vi "温度采集 - TP1.vi"(7 "CSM Name":string="TP1") -> ()   [LabVIEW 2026, in "UI-温度采集.lvlib"]
uses:
  Supports/Sample Settings.ctl
  Supports/Ch Settings.ctl
  Data ColndSave/Supports/Time and Data.ctl
  <userlib>/_NEVSTOP/Communicable State Machine(CSM)/_Polymophic/CSM - Filter Duplicated Lines.vi
  65d0c194-c74c-4b0e-a0ba-0dceafb13ea2.vi
  a3283b4f-3d7d-475f-8286-b95f18be6a9d.vi
  5ee6f246-6564-45f2-9b1c-adf21ebee76f.vi
  67e6e356-fdb8-4529-b23b-6ce46d2feb59.vi
  c25498cf-601b-4c58-9055-343fcb9f8f4a.vi
  c6692627-02fb-4556-9c5d-59e6097d0856.vi
  8c0fc226-3871-4866-9b38-f175316b3ef9.vi
  <vilib>/Analysis/baseanly.llb/Mean (DBL).vi
  f7ac7929-c03e-4c45-8e54-d37ffbbe8d04.vi
  8417ea6c-3bd9-4cd5-8933-b29b0935beb3.vi
  c0a7cae7-a94b-4088-a6e9-4f476a10c4ba.vi
  <userlib>/_NEVSTOP/Communicable State Machine(CSM)/_Polymophic/CSM - Replace Marks in Messages.vi
  5163a33a-69e0-492d-a74e-a390bdb1a610.vi
  ba09a988-f7d6-44f3-a6d8-47fd2b4ee3b5.vi
  7fbb40cc-7bce-4797-8461-cf694f50c740.vi
  2b068055-2750-46ca-adeb-001e26472588.vi
  <userlib>/_NEVSTOP/Communicable State Machine(CSM)/AdvanceAPI/CSM - Compact Multiple States.vi
  <userlib>/_NEVSTOP/Communicable State Machine(CSM)/AdvanceAPI/CSM - Break Down Multiple States String.vi
  <userlib>/_NEVSTOP/Communicable State Machine(CSM)/_Shared/Remove Comments from Single-line.vi
  <userlib>/_NEVSTOP/Communicable State Machine(CSM)/_Shared/Split Single-line Message.vi
  <userlib>/_NEVSTOP/Communicable State Machine(CSM)/_Shared/Trim Single-line Text.vi
  <userlib>/_NEVSTOP/Communicable State Machine(CSM)/AdvanceAPI/CSM - Revert Arguments-Safe String.vi
  <userlib>/_NEVSTOP/Communicable State Machine(CSM)/AdvanceAPI/CSM - Make String Arguments Safe.vi
  c25498cf-601b-4c58-9055-343fcb9f8f4a.vi/99de0c97-112a-4c86-9094-c187659127e1.vi
  <userlib>/_NEVSTOP/Communicable State Machine(CSM)/Utility/Build Error Cluster.vi
  c6692627-02fb-4556-9c5d-59e6097d0856.vi/99de0c97-112a-4c86-9094-c187659127e1.vi
  f7ac7929-c03e-4c45-8e54-d37ffbbe8d04.vi/99de0c97-112a-4c86-9094-c187659127e1.vi
  8417ea6c-3bd9-4cd5-8933-b29b0935beb3.vi/99de0c97-112a-4c86-9094-c187659127e1.vi
  <userlib>/_NEVSTOP/Communicable State Machine(CSM)/AdvanceAPI/CSM - Keywords.vi
  <userlib>/_NEVSTOP/Communicable State Machine(CSM)/addons/API-String-Arugments-Support/_Support/Data To API String Arguments.vi
  <userlib>/_NEVSTOP/Communicable State Machine(CSM)/addons/INI-Static-Variable-Support/_Support/instances/_CSM - Read File Logger Configuration - v1.0.vi
  <vilib>/Utility/Data Type/Get Type Information.vi
  <userlib>/_NEVSTOP/Communicable State Machine(CSM)/addons/API-String-Arugments-Support/_Support/Data To SingleElementsArray_csm.vi
  <userlib>/_NEVSTOP/Communicable State Machine(CSM)/addons/INI-Static-Variable-Support/_Support/Parse Used Session and Name.vi
  <userlib>/_NEVSTOP/Communicable State Machine(CSM)/addons/INI-Static-Variable-Support/_Support/INI-FGV(lvlibp).vi
  <userlib>/_NEVSTOP/Communicable State Machine(CSM)/addons/INI-Static-Variable-Support/_Support/Populate String with INI Variable.vi
  <userlib>/_NEVSTOP/Communicable State Machine(CSM)/addons/API-String-Arugments-Support/_Support/Convert API String Arguments to Data(variant).vi
  <userlib>/_NEVSTOP/Communicable State Machine(CSM)/addons/API-String-Arugments-Support/_Support/SingleElementsArray To Data_csm.vi
  <userlib>/_NEVSTOP/Communicable State Machine(CSM)/addons/MassData-Parameter/_support/FGV-MassData(lvlibp).vi
  <userlib>/_NEVSTOP/Communicable State Machine(CSM)/Communicable State Machine.lvlib
  <vilib>/Analysis/NI_AALBase.lvlib
  Acquisition/Acquisition.lvlib
  <userlib>/_NEVSTOP/Communicable State Machine(CSM)/addons/MassData-Parameter/CSM MassData Parameter Support.lvlib
  <userlib>/_NEVSTOP/Communicable State Machine(CSM)/addons/INI-Static-Variable-Support/INI-Static-Variable-Support.lvlib
  <userlib>/_NEVSTOP/Communicable State Machine(CSM)/addons/Watchdog/CSM Watchdog.lvlib
  <userlib>/_NEVSTOP/Communicable State Machine(CSM)/addons/Logger/CSM File Logger.lvlib
  Logging/Logging.lvlib
  Data ColndSave/Data Collection and Save.lvlib
panel:
  in  "停止":bool
  in  "温度显示":T1(tab)
  in  "温度采集开关":bool
  in  "Offset relative to chX":T2(ring)
  out "Final Temp":dbl[](array[numeric]) format="%#.2g"
  in  "USB Port":refnum<visa-resource-name>="COM3"
  in  "Interval(s)":dbl=0.5
  in  "Calib":dbl[](array[numeric])=[0.0, 0.0, 0.0, 0.0, 0.0, 0.0, 0.0, 0.0]
  out "Offset":dbl[](array[numeric]) format="%#.2g"
  in  "Chart Auto Zoom":bool=TRUE
  in  "ChA":T3
  in  "ChB":T3
  in  "ChC":T3
  in  "ChD":T3
  out "Default 2":waveform(dbl)(graph)
  out "Default 1":waveform(dbl)(graph)
  out "Default 4":waveform(dbl)(graph)
  out "Default 3":waveform(dbl)(graph)
  out "Default 6":waveform(dbl)(graph)
  out "Default 5":waveform(dbl)(graph)
  out "Default 8":waveform(dbl)(graph)
  out "Default 7":waveform(dbl)(graph)
  out "Diff 2 (CHC-CHD)":waveform(dbl)(graph)
  out "DIff 1 (ChA-CHB)":waveform(dbl)(graph)
  in  "子程序？":bool
  out "Error Occurred":errorcluster caption="温度采集-错误输出"
  out "State History":string
  # "-"
  # "-"
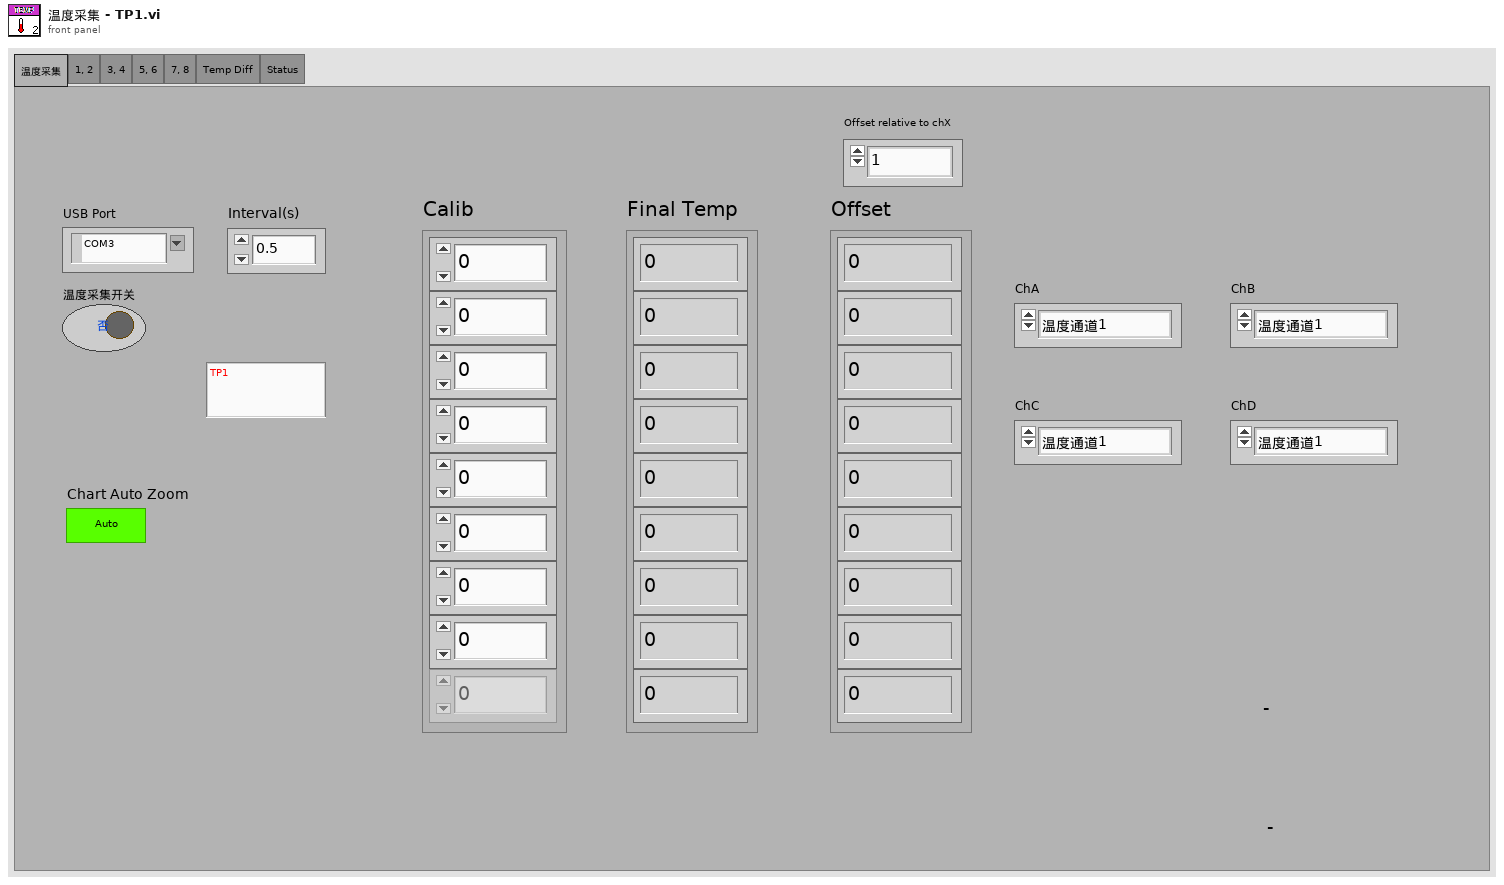
[diagram p1: front panel]
types:
  T1 = enum32{"温度采集", "1, 2", "3, 4", "5, 6", "7, 8", "Temp Diff", "Status"}
  T2 = enum16{"1", "2", "3", "4", "5", "6", "7", "8", "中值", "平均值"}
  T3 = typedef "温度通道索引_全局.ctl" = enum16{"温度通道1", "温度通道2", "温度通道3", "温度通道4", "温度通道5", "温度通道6", "温度通道7", "温度通道8", "TC1控制温度", "TC1实际温度", "TC1实际输出电压", "TC1实际输出电流", "TC1实际输出功率", "TC2控制温度", "TC2实际温度", "TC2实际输出电压", "TC2实际输出电流", "TC2实际输出功率", "压力(电压值)", "压力(g)", "Zolix当前位置", "Zolix速度", "步进电机位置", "步进电机速度", "温度", "湿度"}
  T4 = cluster{"Enable":bool, "Limit":cluster{"FileSize":i64, "FileNum":i32}, "Timestamp.Format":string, "AutoExit":bool}
  T5 = enum32{"Invalid", "Standard", "Closed", "Hidden", "Minimized", "Maximized"}
  T6 = enum32{"invalid app kind", "Development System", "Run Time System", "Student Edition", "Embedded LabVIEW", "Evaluation", "Custom"}
  T7 = typedef "Communicable State Machine.lvlib/_CSM_Response Source Message.ctl" = cluster{"‘State":string, "’Arguments":string, "’Error":errorcluster}
  T8 = cluster{"Current VI Reference":refnum<vi>, "Close Panel on Exit?":bool}
  T9 = typedef "UI-温度采集.lvlib/Sample Settings.ctl" = cluster{"USB Port":refnum<visa-resource-name>, "Interval(s)":dbl, "Calib":dbl[]}
  T10 = typedef "Data Collection and Save.lvlib/Time and Data.ctl" = cluster{"采集时间":timestamp, "Data":dbl[]}
  T11 = cluster{"Core":cluster{"Current VI Reference":refnum<vi>, "Close Panel on Exit?":bool}, "Sample Settings":T9, "Time and Data":T10, "子程序？":bool}
  T12 = typedef "UI-温度采集.lvlib/Ch Settings.ctl" = cluster{"Offset relative to chX":enum16{"1", "2", "3", "4", "5", "6", "7", "8", "中值", "平均值"}, "ChA":T3, "ChB":T3, "ChC":T3, "ChD":T3}
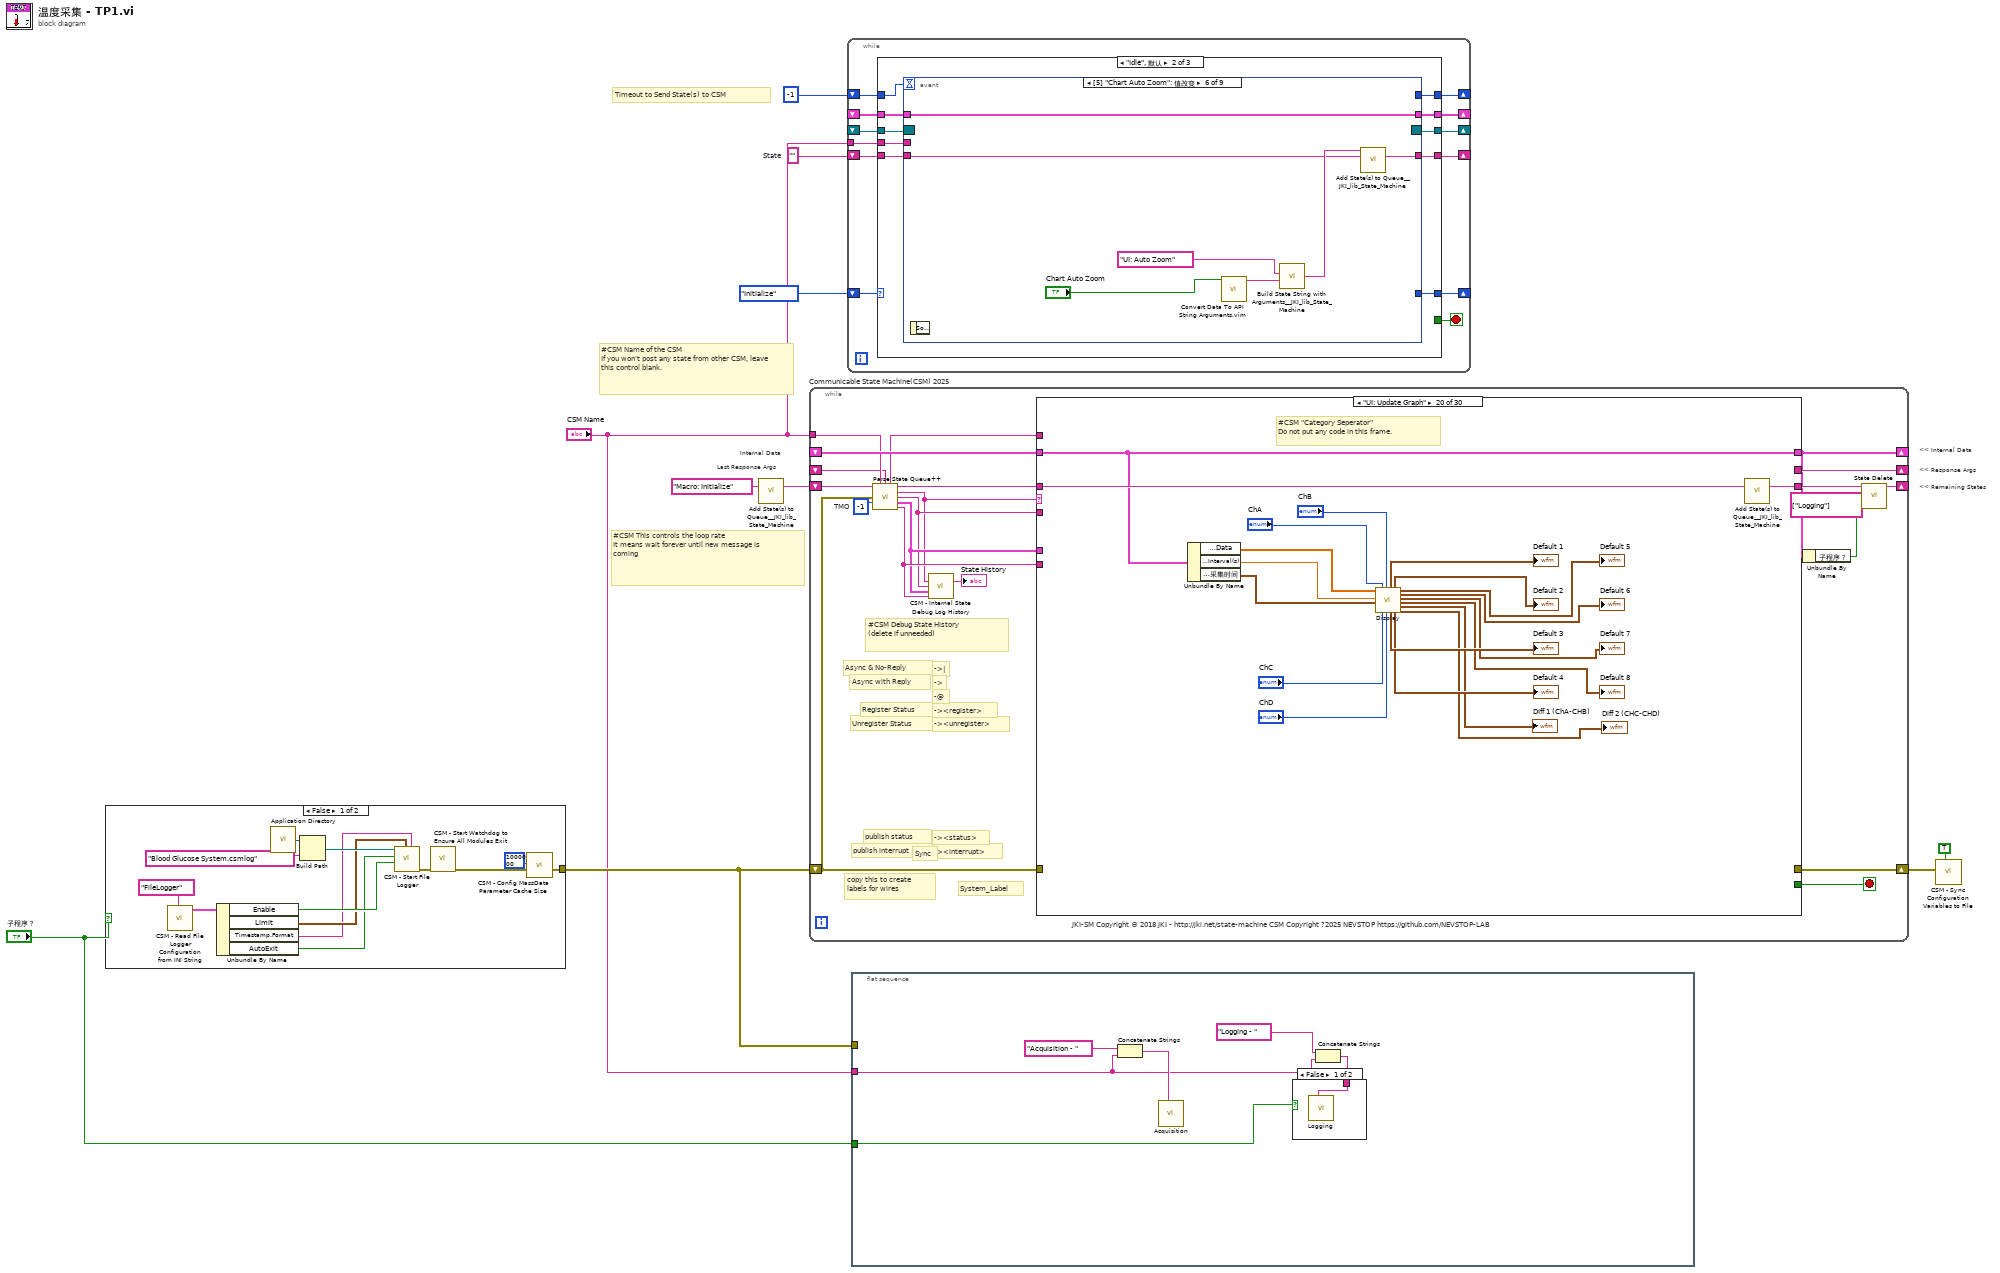
[diagram p0: block diagram]
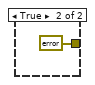
[diagram p2: hidden frame]
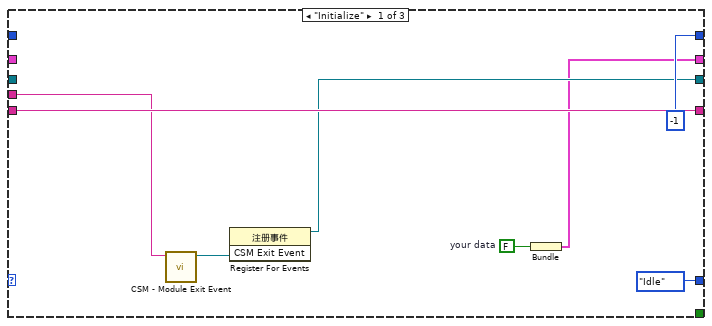
[diagram p4: hidden frame]
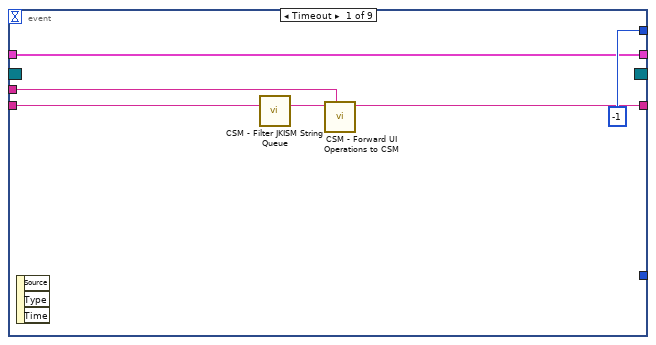
[diagram p5: hidden frame]
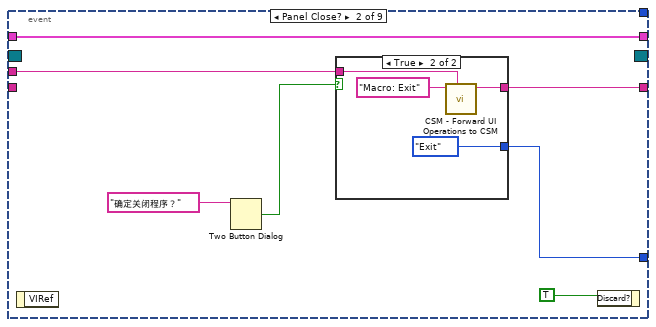
[diagram p6: hidden frame]
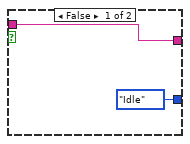
[diagram p7: hidden frame]
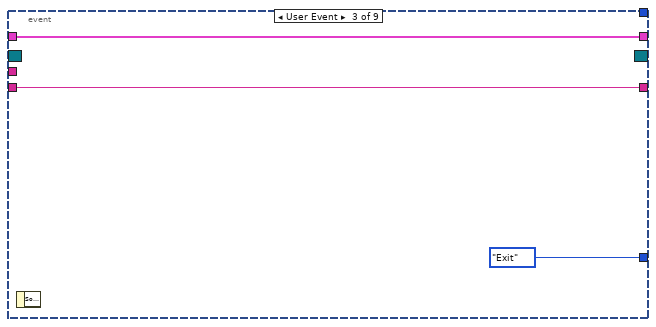
[diagram p8: hidden frame]
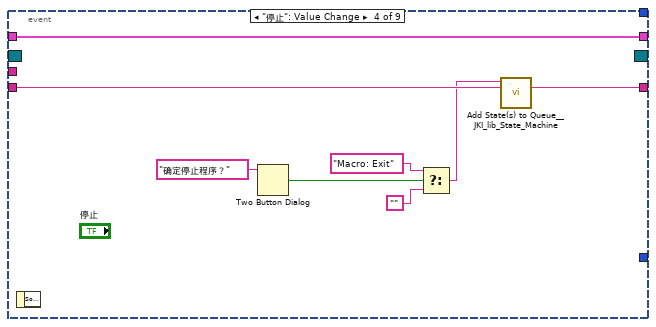
[diagram p9: hidden frame]
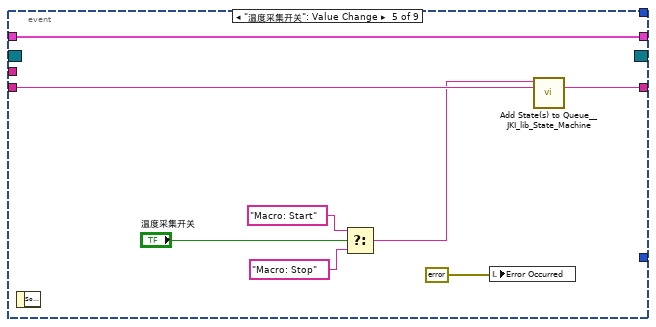
[diagram p10: hidden frame]
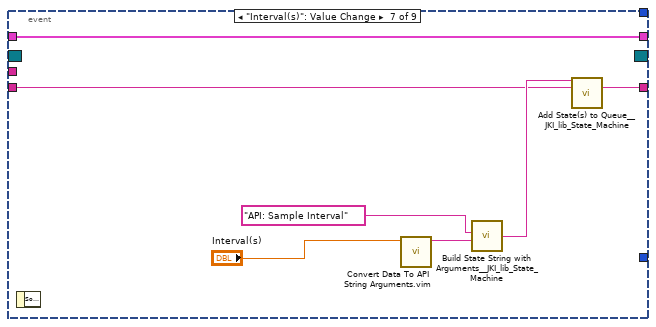
[diagram p11: hidden frame]
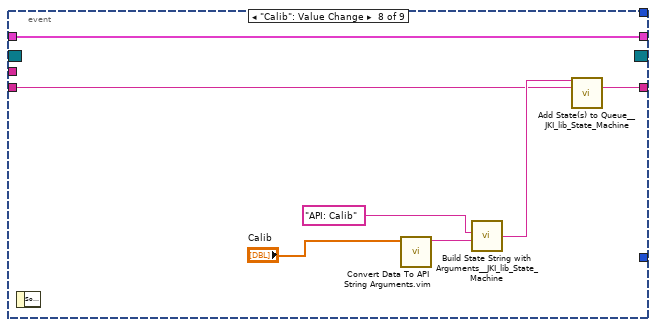
[diagram p12: hidden frame]
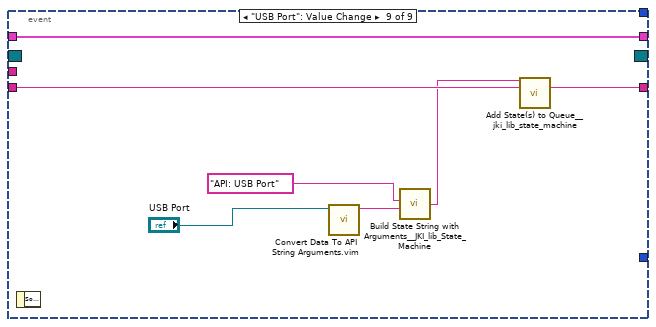
[diagram p13: hidden frame]
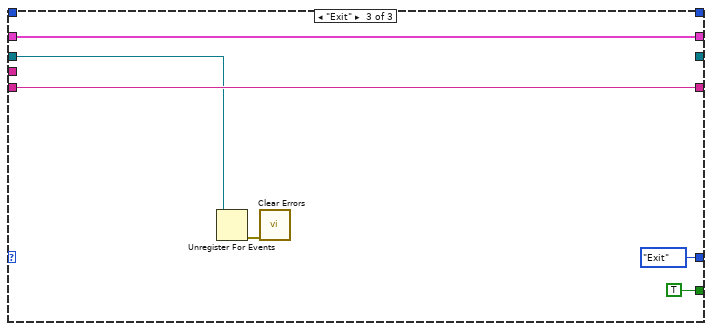
[diagram p14: hidden frame]
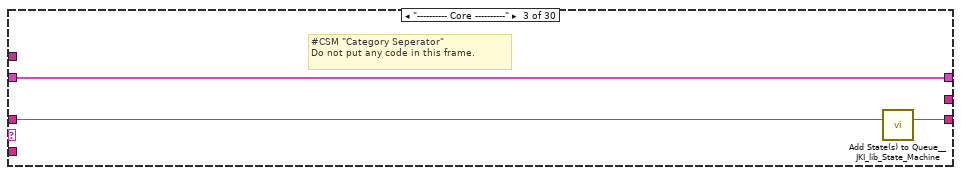
[diagram p17: hidden frame]
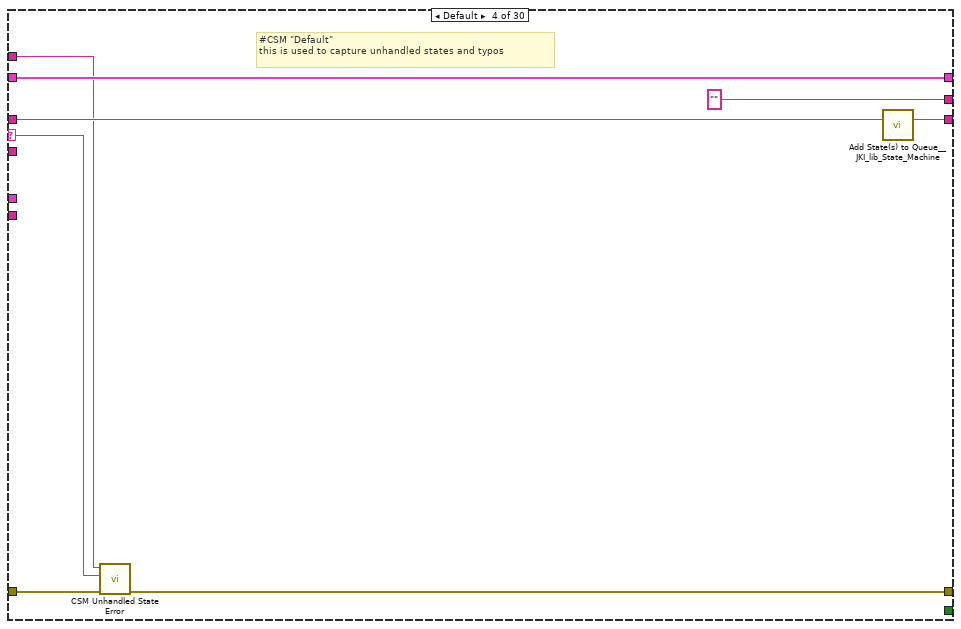
[diagram p18: hidden frame]
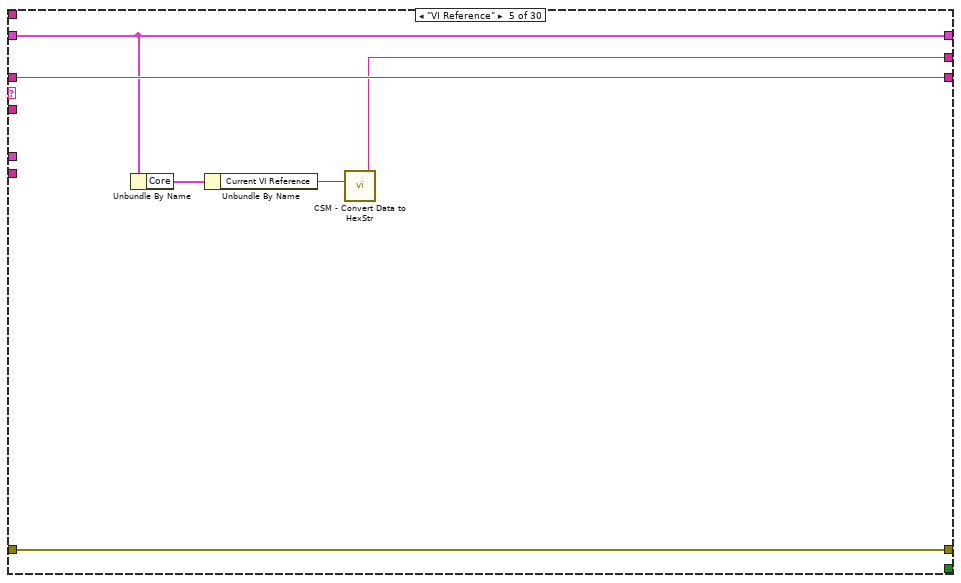
[diagram p19: hidden frame]
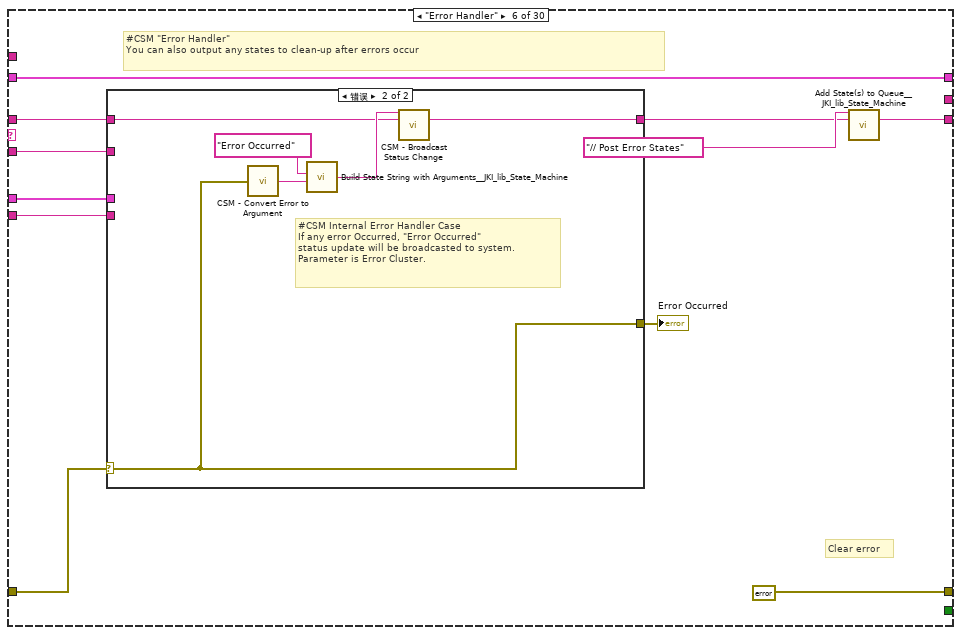
[diagram p20: hidden frame]
diagram:
  w9 = ""  # State
  # "Timeout to Send State(s) to CSM"
  # "Last Response Args"
  # "Internal Data"
  # "#CSM Name of the CSM\nIf you won't post any state from other CSM, leave this control blank."
  # "#CSM This controls the loop rate\nIt means wait forever until new message is coming"
  # "<< Internal Data"
  # "<< Response Args"
  # "<< Remaining States"
  n1 = case shown="False" "子程序？" {
    tunnel: [w11 errorcluster {"status"=FALSE, "code"=0, "source"=""} ("Error out")] -> w5
    frame False {
      n2 = call-poly <userlib>:"CSM - Read File Logger Configuration from INI String.vi"("Section Name(\"FileLogger\")"="FileLogger" ("Section Name(\"\" as Default)")) -> ("FileLogger Configuration-v1"=w18:T4)  [unwired: 7 in, 1 out]
      n3 = Unbundle By Name(w18) -> ("Enable"=w17:bool, "Limit"=w16:cluster{"FileSize":i64, "FileNum":i32}, "Timestamp.Format"=w14:string, "AutoExit"=w15:bool)
      n4 = call <vilib>:"Application Directory.vi"() -> ("Application Directory"=w23:path)
      n5 = Build Path(base path=w23, name or relative path="Blood Glucose System.csmlog") -> (appended path=w21:path)
      n6 = call <userlib>:"CSM - Start File Logger.vi"("Timestamp Format"=w14, "Log Limit"=w16, "Watchdog? (T)"=w17, "Exit When All Module Exist? (F)"=w15, "Log File Path"=w21) -> ("error out"=w20:errorcluster)  [unwired: 4 in, 2 out]
      n7 = call <userlib>:"CSM - Start Watchdog to Ensure All Modules Exit.vi"("error in (no error)"=w20) -> ("error out"=w12:errorcluster)  [unwired: 10 in]
      n8 = call <userlib>:"CSM - Config MassData Parameter Cache Size.vi"("Error in"=w12, "Size (50M)"=1000000 ("size(1M)")) -> ("Error out"=w11:errorcluster)  [unwired: 9 in]
    }
    frame True {
    }
  }
  n9 = call <vilib>:"Add State(s) to Queue__JKI_lib_State_Machine.vi"("State(s) in (\"\")"="Macro: Initialize" ("Init State(\"Macro: Initialize\")")) -> ("States Out"=w6:string)  [unwired: 14 in]
  n10 = while "Communicable State Machine(CSM) 2025" {
    shift-right: [w26] -> _
    shift-left: _ -> [w41]
    shift-right: [w43] -> w3
    shift-left: w5 -> [w31]
    shift-right: [w28] -> _
    shift-left: w6 -> [w44]
    tunnel: "CSM Name" -> [w38]
    shift-right: [w39] -> _
    shift-left: _ -> [w33]
    stop <- w42 stop-if-true
    w40 = -1  # TMO
    # "#CSM Debug State History\n(delete if unneeded)"
    # "-><interrupt>"
    # "-><status>"
    # "-><unregister>"
    # "-><register>"
    # "-@"
    # "->"
    # "->|"
    # "publish interrupt"
    # "publish status"
    # "Unregister Status"
    # "Register Status"
    # "Sync"
    # "Async with Reply"
    # "Async & No-Reply"
    # "JKI-SM Copyright © 2018 JKI - http://jki.net/state-machine CSM Copyright ?2025 NEVSTOP https://github.com/NEVSTOP-LAB"
    # "copy this to create labels for wires"
    # "System_Label"
    n11 = call <userlib>:"Parse State Queue++.vi"("State Queue"=w44, "Name (\"\" to Use UUID)"=w38, "Response Arguments"=w33, "Previous Error"=w31, "Dequeue (1 ms)"=w40) -> ("Name Used"=w32:string, "Remaining States"=w45:string, "Current State"=w34:string, "Arguments"=w35:string, "Additional Information"=w36:T7, "Source CSM"=w37:string)  [unwired: 5 in]
    n12 = call <userlib>:"CSM - Internal State Debug Log History.vi"("State"=w34, "Arguments (\"\")"=w35, ">> Response Source Message >>"=w36, "Source (\"\")"=w37) -> ("Debug Log"=→"State History":string)  [unwired: 11 in]
    n13 = case shown="\"UI: Update Graph\"" w34 {
      selector: w34 -> [_ _ _ w56 _ _ _ _ _ _ _ _ _ _ _ _ _ _ _ _ _ _ _ _ _ _ _ _ _ _]
      tunnel: w45 -> [w46 w49 w52 w60 w65 w71 w96 w102 w108 w118 w125 w137 w141 w144 w164 w176 w223 w226 w237 w257 w264 w269 w275 w284 w291 w297 w300 w311 w321 w328]
      tunnel: w35 -> [_ _ _ _ _ w70 w92 w99 w105 w112 _ _ _ _ _ w171 _ _ _ _ w260 _ _ _ _ _ _ w306 w314 w324]
      tunnel: w41 -> [w47 w48 w50 w58 w64 w76 w94 w100 w106 w116 w124 w131 w139 w142 _ w168 w218 w224 w227 w255 w262 w267 w273 w281 w289 w295 w302 w307 w316 w326]
      tunnel: [_ _ _ w53 w66 errorcluster {"status"=FALSE, "code"=0, "source"=""} ("error out") w89 w97 w103 w119 _ _ _ _ _ _ w219 _ _ _ _ _ _ _ _ _ _ _ _ _] -> w43
      tunnel: w31 -> [_ _ _ w54 w66 w74 w90 w98 w104 _ _ _ _ _ _ _ w220 _ _ _ _ _ _ _ _ _ _ _ _ _]
      tunnel: [w46 w49 w51 w59 w65 w72 w95 w101 w107 w117 w125 w136 w140 w143 w163 w175 w222 w225 w236 w256 w263 w268 w274 w283 w290 w296 w301 w312 w322 w329] -> w29
      tunnel: [_ _ _ _ _ _ TRUE _ _ _ _ _ TRUE _ _ _ _ _ _ _ _ _ _ _ _ _ _ _ _ _] -> w42
      tunnel: [w47 w48 w50 w58 w64 w76 w94 w100 w106 w115 w124 w135 w139 w142 w162 w165 w218 w224 w227 w255 w262 w267 w273 w281 w289 w295 w302 w303 w315 w325] -> w26
      tunnel: w37 -> [_ _ _ _ _ w69 _ _ _ w113 _ _ _ _ _ _ _ _ _ _ _ _ _ _ _ _ _ _ _ _]
      tunnel: w36 -> [_ _ _ _ _ w68 _ _ _ w114 _ _ _ _ _ _ _ _ _ _ _ _ _ _ _ _ _ _ _ _]
      tunnel: [_ _ _ "" w61 _ _ _ _ _ _ _ _ _ _ _ _ _ _ _ _ _ _ _ _ _ _ _ _ _] -> w39
      tunnel: w32 -> [_ _ _ w55 _ _ w91 _ _ _ _ _ _ _ w157 _ w215 _ _ _ _ _ w271 w278 w287 w293 _ w309 w319 _]
      frame "", "Idle" {
        # "#CSM \"Idle/Event Handler\"\nexecutes when the state queue is empty"
      }
      frame "CSM Documentation" {
        # "#CSM State Syntax\n\n// Comment line, all text to the right of “//” will be ignored\n// Local Message Example\nDoSth: DoA >> Arguments\n\n// Sync Call Example\nAPI: xxxx >> Arguments -@ TargetModule\n\n// Async Call Example\nAPI: xxxx >> Arguments -> TargetModule\n\n// Async Call without Reply Example\nAPI: xxxx >> Arguments ->| TargetModule\n\n// Broadcast normal status:\nStatus >> StatusArguments  -><status>\n\n// Broadcast Interrupt status:\nInterrupt >> StatusArguments  -><interrupt>\n\n// Register Source Module's status to Handler Module\nStatus@Source Module >> Handler Module@Handler Module -><register>\n\n// Unegister Source Module's status\nStatus@Source Module >> Handler Module -><unregister>"
        # "#CSM README FIRST\n\nCommunicable State Machine(CSM) is a LabVIEW application framework that builds upon JKI State Machine(JKISM). It follows the pattern of JKISM and extends the keywords to describe message communication between modules, including concepts such as Sync-Message, Async-Message, Subscription/Unsubscription of status - essential elements for creating reusable code modules. For more information, please visit the CSM wiki: https://nevstop-lab.github.io/CSM-Wiki/\n\nFor instructions on JKI State Machine, visit: \n    http://jki.net/state-machine/\nFor information about CSM, visit: \n    https://github.com/NEVSTOP-LAB"
        # "#CSM \"Documentation\"\nCase for holding CSM Documenation"
      }
      frame "---------- Core ----------" {
        # "#CSM \"Category Seperator\"\nDo not put any code in this frame."
        n14 = call <vilib>:"Add State(s) to Queue__JKI_lib_State_Machine.vi"("State(s) in (\"\")"=w52) -> ("States Out"=w51:string)  [unwired: 14 in]
      }
      frame Default {
        # "#CSM \"Default\"\nthis is used to capture unhandled states and typos"
        n15 = call <userlib>:"CSM Unhandled State Error.vi"("error in (no error)"=w54, "Undefined State"=w56, "CSM Name"=w55) -> ("error out"=w53:errorcluster)  [unwired: 8 in]
        n16 = call <vilib>:"Add State(s) to Queue__JKI_lib_State_Machine.vi"("State(s) in (\"\")"=w60) -> ("States Out"=w59:string)  [unwired: 14 in]
      }
      frame "VI Reference" {
        n17 = Unbundle By Name(w64) -> ("Core"=w63:T8)
        n18 = Unbundle By Name(w63) -> ("Current VI Reference"=w62:refnum<vi>)
        n19 = call <userlib>:"CSM - Convert Data to HexStr.vi"("Variant"=w62) -> ("HEX String (0-9,A-F)"=w61:string)  [unwired: 8 in]
      }
      frame "Error Handler" {
        # "#CSM \"Error Handler\"\nYou can also output any states to clean-up after errors occur"
        # "Clear error"
        n20 = case shown="错误" w74 {
          selector: w74 -> [_ w83]
          tunnel: [w81 w85] -> w73
          tunnel: w71 -> [w81 w84]
          tunnel: w70 -> [w80 _]
          tunnel: w69 -> [_ _]
          tunnel: w68 -> [_ _]
          tunnel: [w78 w83] -> w67
          frame No Error {
            n21 = call <userlib>:"CSM - Convert Argument to Error.vi"("Argument"=w80) -> ("Error"=w79:errorcluster)  [unwired: 4 in]
            n22 = flat-sequence {
              tunnel: w79 -> [w82]
              tunnel: [w82] -> w78
              frame #0 {
              }
            }
          }
          frame Error {
            # "#CSM Internal Error Handler Case \nIf any error Occurred, \"Error Occurred\" \nstatus update will be broadcasted to system.\nParameter is Error Cluster."
            n23 = call <userlib>:"CSM - Convert Error to Argument.vi"("Error"=w83) -> ("Argument"=w87:string)  [unwired: 4 in]
            n24 = call <vilib>:"Build State String with Arguments__JKI_lib_State_Machine.vi"("Arguments (\"\")"=w87, "State"="Error Occurred" ("Status with Arguments")) -> ("State with Arguments"=w86:string)  [unwired: 4 in]
            n25 = call <userlib>:"CSM - Broadcast Status Change.vi"("Status With Arguments"=w86, "State Queue"=w84) -> ("Remaining States"=w85:string)  [unwired: 13 in]
          }
        }
        "Error Occurred" <- w67
        n26 = call <vilib>:"Add State(s) to Queue__JKI_lib_State_Machine.vi"("State(s) in Front (\"\")"="// Post Error States", "State(s) in (\"\")"=w73) -> ("States Out"=w72:string)  [unwired: 13 in]
      }
      frame "Critical Error" {
        # "#CSM \"Critical Error\"\nWhen any un-recoverable error occurs, CSM goes into this case."
        # "#CSM Stop in Critical Error\nWhen Critical Error occurs, Stop the loop immediately. Do NOT change this unless you fully understand the impact."
        n27 = call <userlib>:"CSM Critical Error.vi"("error in (no error)"=w90, "Arugments (As Reason)"=w92, "CSM Name"=w91) -> ("error out"=w89:errorcluster)  [unwired: 8 in]
        n28 = call <vilib>:"Add State(s) to Queue__JKI_lib_State_Machine.vi"("State(s) in (\"\")"=w96) -> ("States Out"=w95:string)  [unwired: 14 in]
      }
      frame "Target Timeout Error" {
        # "#CSM \"Target Timeout Error\"\nWhen This CSM could not get the sync-call response in time, This CSM goes into this case."
        n29 = call <userlib>:"CSM Target Timeout Error.vi"("error in (no error)"=w98, "Arguments (As CSM Name)"=w99) -> ("error out"=w97:errorcluster)  [unwired: 9 in]
        n30 = call <vilib>:"Add State(s) to Queue__JKI_lib_State_Machine.vi"("State(s) in (\"\")"=w102) -> ("States Out"=w101:string)  [unwired: 14 in]
      }
      frame "Target Error" {
        # "#CSM \"Target Error\"\nWhen This CSM try to communicate with an un-existed CSM, This CSM goes into this case."
        n31 = call <userlib>:"CSM Target Error.vi"("error in (no error)"=w104, "Arguments (As CSM Name)"=w105) -> ("error out"=w103:errorcluster)  [unwired: 9 in]
        n32 = call <vilib>:"Add State(s) to Queue__JKI_lib_State_Machine.vi"("State(s) in (\"\")"=w108) -> ("States Out"=w107:string)  [unwired: 14 in]
      }
      frame "Async Response", "Response" {
        n33 = Unbundle(w114) -> ("‘State"=w111:string, "’Arguments"=w110:string, "’Error"=w109:errorcluster)
        n34 = case shown="默认" w111 {
          tunnel: [w120] -> w117
          tunnel: w118 -> [w121]
          tunnel: [w123] -> w115
          tunnel: w116 -> [w123]
          tunnel: [w122] -> w119
          tunnel: w109 -> [w122]
          tunnel: w113 -> [_]
          tunnel: w112 -> [_]
          tunnel: w110 -> [_]
          frame 默认 {
            # "#CSM \"Async Response\"\nHandle Async-call Response (\"Async Response\" for ->)"
            # "#CSM \"Response\"\nHandle Sync-call Response (\"Response\" for -@)"
            # "#CSM Response Comments\nAfter Message is executed, CSM goes to this state for receive the response.\n    For Async Message(->), \"Async Response\" is used. This CSM will goes to \"Async Message Posted\" immediately and receive the \"Async Response\" after the callee finishes the message.\n    For Sync Message(@),  This CSM will wait until the message is done and immediately goes to \"Response\""
            n35 = call <vilib>:"Add State(s) to Queue__JKI_lib_State_Machine.vi"("State(s) in (\"\")"=w121) -> ("States Out"=w120:string)  [unwired: 14 in]
          }
        }
      }
      frame "Async Message Posted" {
        # "#CSM \"Async Message Posted\"\nAfter Async Message is posted (-> or ->| ), CSM goes to this state for post-action.\nYou can use Argument - State to tell which Async Message is called."
      }
      frame "Initialize Core Data" {
        # "#CSM \"Initialize Core Data\"\nThis is used to determine panel behavior on exit"
        # "originally closed?"
        # "exe?"
        # "If panel starts closed or is an EXE, then close it when we exit"
        n36 = property class="VI"() -> ("FP.State"=w128:T5)  [unwired: 2 in, 2 out]
        n37 = property class="App"() -> ("App.Kind"=w134:T6)  [unwired: 2 in, 2 out]
        n38 = control-ref of="Current VI Reference"() -> (w129:refnum<vi>)
        n39 = Equal?(x=w128, y=T5."Closed" ("Front Panel Window:State")) -> (x = y?=w126:bool)
        n40 = Equal?(x=w134, y=T6."Run Time System" ("Application:Kind")) -> (x = y?=w132:bool)
        n41 = Or(x=w126, y=w132) -> (x .or. y?=w130:bool)
        n42 = Bundle By Name(cluster=w131, "Core.Current VI Reference"=w129, "Core.Close Panel on Exit?"=w130) -> (w135:T11)
        n43 = call <vilib>:"Add State(s) to Queue__JKI_lib_State_Machine.vi"("State(s) in (\"\")"=w137) -> ("States Out"=w136:string)  [unwired: 14 in]
      }
      frame "Exit" {
        # "#CSM \"Exit\"\nCase for exiting the loop. No errors that occur here will be handled."
        n44 = call <vilib>:"Add State(s) to Queue__JKI_lib_State_Machine.vi"("State(s) in (\"\")"=w141) -> ("States Out"=w140:string)  [unwired: 14 in]
      }
      frame "---------- Data ----------" {
        # "#CSM \"Category Seperator\"\nDo not put any code in this frame."
        n45 = call <vilib>:"Add State(s) to Queue__JKI_lib_State_Machine.vi"("State(s) in (\"\")"=w144) -> ("States Out"=w143:string)  [unwired: 14 in]
      }
      frame "Data: Initialize" {
        w150 = T10 {"采集时间"=timestamp(0 s since 1904-01-01), "Data"=[0.0, 0.0, 0.0, 0.0, 0.0, 0.0, 0.0, 0.0]}  # Time and Data
        w153 = T12 {"Offset relative to chX"=enum."1", "ChA"=enum."温度通道1", "ChB"=enum."温度通道1", "ChC"=enum."温度通道1", "ChD"=enum."温度通道1"}  # Ch Settings
        w146 = T9 {"USB Port"="COM3", "Interval(s)"=0.5, "Calib"=[0.0, 0.0, 0.0, 0.0, 0.0, 0.0, 0.0, 0.0]}  # Sample Settings
        w161 = T8 {"Current VI Reference"=refnum, "Close Panel on Exit?"=FALSE}  # Core
        # "#CSM \"Data: Initialize\"\nInitialize the shift-register data, here.\n(data names are defined by what you wire into the bundle function)"
        # "#CSM do not delete - used by framework"
        # "#CSM Add new data here."
        # "#CSM Data names and types of shift register data are defined by this bundle."
        n46 = local read "子程序？"() -> (w149:bool)
        n47 = call "CSM - Read Cluster Elements From Session.vim"("Section Name (\"\" as Default)"=w157, "Cluster"=w153) -> ("Cluster out"=w158:T12)  [unwired: 6 in, 1 out]
        n48 = local write "温度采集开关"(FALSE ("温度采集开关")) -> ()
        n49 = call "CSM - Read Cluster Elements From Session.vim"("Section Name (\"\" as Default)"=w157, "Cluster"=w146) -> ("Cluster out"=w147:T9)  [unwired: 6 in, 1 out]
        n50 = Unbundle By Name(w158) -> ("Offset relative to chX"=w156:T2, "ChA"=w155:T3, "ChB"=w154:T3, "ChC"=w152:T3, "ChD"=w151:T3)
        n51 = local write "Error Occurred"(errorcluster {"status"=FALSE, "code"=0, "source"=""} ("Error Occurred")) -> ()
        n52 = Select(t=w147, s=TRUE, f=w146) -> (s? t:f=w145:T9)
        n53 = local write "ChA"(w155) -> ()
        n54 = local write "ChB"(w154) -> ()
        n55 = local write "ChC"(w152) -> ()
        n56 = local write "ChD"(w151) -> ()
        n57 = local write "Offset relative to chX"(w156) -> ()
        n58 = Bundle("Core"=w161, "Sample Settings"=w145, "Time and Data"=w150, "子程序？"=w149) -> (w162:T11)  [unwired: 1 in]
        n59 = call <vilib>:"Add State(s) to Queue__JKI_lib_State_Machine.vi"("State(s) in (\"\")"=w164) -> ("States Out"=w163:string)  [unwired: 14 in]
      }
      frame "Data: Update Indicators" {
        w169 = T10 {"采集时间"=timestamp(0 s since 1904-01-01), "Data"=[]}  # Time and Data
        n60 = call "CSM - Convert Argument to MassData.vim"("Type"=w169, "MassData Argument"=w171) -> ("Data"=w170:T10)  [unwired: 6 in, 1 out]
        n61 = Unbundle By Name(w170) -> ("采集时间"=w167:timestamp, "Data"=w166:dbl[])
        "Final Temp" <- w166
        n62 = in-place {
          in-place-border: w167 -> [w179]
          in-place-border: w166 -> [w178]
          n63 = in-place-cluster #1(w168) -> ()  [unwired: 2 out]
          n64 = in-place-cluster #1("Time and Data.采集时间"=w179, "Time and Data.Data"=w178) -> (w165:T11)
        }
        n65 = case shown="\"2\"" "Offset relative to chX" {
          selector: "Offset relative to chX" -> [w180 w184 w187 w189 w192 w196 w198 w202 _ _]
          tunnel: w166 -> [w182 w183 w188 w190 w194 w197 w199 w203 w205 w206]
          tunnel: [w181 w185 w186 w191 w193 w195 w200 w201 w204 w207] -> w173
          frame "1" {
            n66 = Index Array(array=w182, index=w180) -> (element=w181:dbl)
          }
          frame "2" {
            n67 = Index Array(array=w183, index=w184) -> (element=w185:dbl)
          }
          frame "3" {
            n68 = Index Array(array=w188, index=w187) -> (element=w186:dbl)
          }
          frame "4" {
            n69 = Index Array(array=w190, index=w189) -> (element=w191:dbl)
          }
          frame "5" {
            n70 = Index Array(array=w194, index=w192) -> (element=w193:dbl)
          }
          frame "6" {
            n71 = Index Array(array=w197, index=w196) -> (element=w195:dbl)
          }
          frame "7" {
            n72 = Index Array(array=w199, index=w198) -> (element=w200:dbl)
          }
          frame "8" {
            n73 = Index Array(array=w203, index=w202) -> (element=w201:dbl)
          }
          frame "中值" {
            n74 = call <vilib>:"Median.vi"("X"=w205) -> ("median"=w204:dbl)  [unwired: 1 out]
          }
          frame "平均值" {
            n75 = call-poly <vilib>:"Mean.vi"("X"=w206) -> ("mean"=w207:dbl)  [unwired: 1 out]
          }
        }
        n76 = Subtract(x=w166, y=w173) -> (x-y=→"Offset":dbl[])
        n77 = call <vilib>:"Add State(s) to Queue__JKI_lib_State_Machine.vi"("State(s) in Front (\"\")"="UI: Update Graph" ("State(s) in Front (\"\")"), "State(s) in (\"\")"=w176) -> ("States Out"=w175:string)  [unwired: 13 in]
      }
      frame "Data: Cleanup" {
        w214 = T12 {"Offset relative to chX"=enum."1", "ChA"=enum."温度通道1", "ChB"=enum."温度通道1", "ChC"=enum."温度通道1", "ChD"=enum."温度通道1"}  # Ch Settings
        # "#CSM \"Data: Cleanup\"\nCleanup any data and references, here.\n(this is called automatically, by the Macro: Exit)"
        n78 = local read "ChA"() -> (w212:T3)
        n79 = local read "ChB"() -> (w211:T3)
        n80 = local read "ChC"() -> (w210:T3)
        n81 = local read "ChD"() -> (w209:T3)
        n82 = Unbundle By Name(w218) -> ("Core.Current VI Reference"=w221:refnum<vi>, "Sample Settings"=w216:T9)
        n83 = local read "Offset relative to chX"() -> (w213:T2)
        n84 = Bundle By Name(cluster=w214, "Offset relative to chX"=w213, "ChA"=w212, "ChB"=w211, "ChC"=w210, "ChD"=w209) -> (w208:T12)
        n85 = call "CSM - Write Configuration Variable.vim"("Section Name (\"\" as Default)"=w215, "Configuration"=w216) -> ()  [unwired: 6 in, 2 out]
        n86 = call "CSM - Write Configuration Variable.vim"("Section Name (\"\" as Default)"=w215, "Configuration"=w208) -> ()  [unwired: 6 in, 2 out]
        n87 = Close Reference(reference=w221, error in (no error)=w220) -> (error out=w219:errorcluster)
        n88 = local write "温度采集开关"(FALSE ("温度采集开关")) -> ()
        n89 = call <vilib>:"Add State(s) to Queue__JKI_lib_State_Machine.vi"("State(s) in (\"\")"=w223) -> ("States Out"=w222:string)  [unwired: 14 in]
      }
      frame "---------- UI ----------" {
        # "#CSM \"Category Seperator\"\nDo not put any code in this frame."
        n90 = call <vilib>:"Add State(s) to Queue__JKI_lib_State_Machine.vi"("State(s) in (\"\")"=w226) -> ("States Out"=w225:string)  [unwired: 14 in]
      }
      frame "UI: Initialize" {
        w234 = u8 2 ("X标尺.标尺调节")
        w235 = waveform(dbl)[] [] ("历史数据")
        # "#CSM \"Category Seperator\"\nDo not put any code in this frame."
        n91 = Unbundle By Name(w227) -> ("Time and Data.Data"=w233:dbl[], "Sample Settings.USB Port"=w231:refnum<visa-resource-name>, "Sample Settings.Interval(s)"=w230:dbl, "Sample Settings.Calib"=w229:dbl[], "子程序？"=w228:bool)
        n92 = Not(x=w228) -> (.not. x?=w232:bool)
        n93 = property on="停止" class="Bool"("Visible"=w232) -> ()  [unwired: 2 in, 2 out]
        n94 = local write "Calib"(w229) -> ()
        n95 = local write "USB Port"(w231) -> ()
        n96 = local write "Interval(s)"(w230) -> ()
        n97 = local write "Final Temp"(w233) -> ()
        n98 = local write "Offset"(w233) -> ()
        n99 = property on="Default 1" class="WFChart (严格)"("History Data"=w235) -> ()  [unwired: 2 in, 2 out]
        n100 = property on="Default 2" class="WFChart (严格)"("History Data"=w235) -> ()  [unwired: 2 in, 2 out]
        n101 = property on="Default 3" class="WFChart (严格)"("History Data"=w235) -> ()  [unwired: 2 in, 2 out]
        n102 = property on="Default 4" class="WFChart (严格)"("History Data"=w235) -> ()  [unwired: 2 in, 2 out]
        n103 = property on="DIff 1 (ChA-CHB)" class="WFChart (严格)"("History Data"=w235) -> ()  [unwired: 2 in, 2 out]
        n104 = property on="Default 5" class="WFChart (严格)"("History Data"=w235) -> ()  [unwired: 2 in, 2 out]
        n105 = property on="Default 6" class="WFChart (严格)"("History Data"=w235) -> ()  [unwired: 2 in, 2 out]
        n106 = property on="Default 7" class="WFChart (严格)"("History Data"=w235) -> ()  [unwired: 2 in, 2 out]
        n107 = property on="Default 8" class="WFChart (严格)"("History Data"=w235) -> ()  [unwired: 2 in, 2 out]
        n108 = property on="Diff 2 (CHC-CHD)" class="WFChart (严格)"("History Data"=w235) -> ()  [unwired: 2 in, 2 out]
        n109 = property on="Default 1" class="WFChart (严格)"("XScale.ScaleFit"=w234) -> ()  [unwired: 2 in, 2 out]
        n110 = property on="Default 2" class="WFChart (严格)"("XScale.ScaleFit"=w234) -> ()  [unwired: 2 in, 2 out]
        n111 = property on="DIff 1 (ChA-CHB)" class="WFChart (严格)"("XScale.ScaleFit"=w234) -> ()  [unwired: 2 in, 2 out]
        n112 = property on="Default 3" class="WFChart (严格)"("XScale.ScaleFit"=w234) -> ()  [unwired: 2 in, 2 out]
        n113 = property on="Default 4" class="WFChart (严格)"("XScale.ScaleFit"=w234) -> ()  [unwired: 2 in, 2 out]
        n114 = property on="Default 5" class="WFChart (严格)"("XScale.ScaleFit"=w234) -> ()  [unwired: 2 in, 2 out]
        n115 = property on="Default 6" class="WFChart (严格)"("XScale.ScaleFit"=w234) -> ()  [unwired: 2 in, 2 out]
        n116 = property on="Default 7" class="WFChart (严格)"("XScale.ScaleFit"=w234) -> ()  [unwired: 2 in, 2 out]
        n117 = property on="Default 8" class="WFChart (严格)"("XScale.ScaleFit"=w234) -> ()  [unwired: 2 in, 2 out]
        n118 = property on="Diff 2 (CHC-CHD)" class="WFChart (严格)"("XScale.ScaleFit"=w234) -> ()  [unwired: 2 in, 2 out]
        n119 = call <vilib>:"Add State(s) to Queue__JKI_lib_State_Machine.vi"("State(s) in (\"\")"=w237) -> ("States Out"=w236:string)  [unwired: 14 in]
      }
      frame "UI: Update Graph" {
        # "#CSM \"Category Seperator\"\nDo not put any code in this frame."
        n120 = Unbundle By Name(w255) -> ("Time and Data.Data"=w254:dbl[], "Sample Settings.Interval(s)"=w253:dbl, "Time and Data.采集时间"=w238:timestamp)
        n121 = call "Display.vi"("Data"=w254, "dt"=w253, "t0"=w238, "索引 1"="ChA", "索引 3"="ChC", "索引 2"="ChB", "索引 4"="ChD") -> ("输出波形 1"=→"Default 1":waveform(dbl), "输出波形 3"=→"Default 3":waveform(dbl), "输出波形 2"=→"Default 2":waveform(dbl), "输出波形 4"=→"Default 4":waveform(dbl), "输出波形 5"=→"Default 5":waveform(dbl), "输出波形 6"=→"Default 6":waveform(dbl), "输出波形 7"=→"Default 7":waveform(dbl), "输出波形 8"=→"Default 8":waveform(dbl), "输出波形 Ch1"=→"DIff 1 (ChA-CHB)":waveform(dbl), "输出波形 Ch2"=→"Diff 2 (CHC-CHD)":waveform(dbl))  [unwired: 3 in]
        n122 = call <vilib>:"Add State(s) to Queue__JKI_lib_State_Machine.vi"("State(s) in (\"\")"=w257) -> ("States Out"=w256:string)  [unwired: 14 in]
      }
      frame "UI: Auto Zoom" {
        # "#CSM \"Category Seperator\"\nDo not put any code in this frame."
        n123 = call "Convert API String Arguments to Data.vim"("Reference Type"=FALSE ("Chart Auto Zoom"), "API String"=w260) -> ("Data"=w259:bool)  [unwired: 6 in, 1 out]
        n124 = case shown="False" w259 {
          tunnel: [u8 0 ("X标尺.标尺调节") u8 2 ("X标尺.标尺调节")] -> w258
          frame False {
          }
          frame True {
          }
        }
        n125 = property on="Default 1" class="WFChart (严格)"("XScale.ScaleFit"=w258) -> ()  [unwired: 2 in, 2 out]
        n126 = property on="Default 2" class="WFChart (严格)"("XScale.ScaleFit"=w258) -> ()  [unwired: 2 in, 2 out]
        n127 = property on="DIff 1 (ChA-CHB)" class="WFChart (严格)"("XScale.ScaleFit"=w258) -> ()  [unwired: 2 in, 2 out]
        n128 = property on="Default 3" class="WFChart (严格)"("XScale.ScaleFit"=w258) -> ()  [unwired: 2 in, 2 out]
        n129 = property on="Default 4" class="WFChart (严格)"("XScale.ScaleFit"=w258) -> ()  [unwired: 2 in, 2 out]
        n130 = property on="Default 5" class="WFChart (严格)"("XScale.ScaleFit"=w258) -> ()  [unwired: 2 in, 2 out]
        n131 = property on="Default 6" class="WFChart (严格)"("XScale.ScaleFit"=w258) -> ()  [unwired: 2 in, 2 out]
        n132 = property on="Default 7" class="WFChart (严格)"("XScale.ScaleFit"=w258) -> ()  [unwired: 2 in, 2 out]
        n133 = property on="Default 8" class="WFChart (严格)"("XScale.ScaleFit"=w258) -> ()  [unwired: 2 in, 2 out]
        n134 = property on="Diff 2 (CHC-CHD)" class="WFChart (严格)"("XScale.ScaleFit"=w258) -> ()  [unwired: 2 in, 2 out]
        n135 = call <vilib>:"Add State(s) to Queue__JKI_lib_State_Machine.vi"("State(s) in (\"\")"=w264) -> ("States Out"=w263:string)  [unwired: 14 in]
      }
      frame "---------- Macro ----------" {
        # "#CSM \"Category Seperator\"\nDo not put any code in this frame."
        n136 = call <vilib>:"Add State(s) to Queue__JKI_lib_State_Machine.vi"("State(s) in (\"\")"=w269) -> ("States Out"=w268:string)  [unwired: 14 in]
      }
      frame "Macro: Initialize" {
        w272 = "Data: Initialize\nInitialize Core Data\nUI: Initialize\n\n//Permanent registrations\nAcquired Data@Acquisition - <1> >> Data: Update Indicators -><register>\nAcquired Data@Acquisition - <1> >> API: Log@Logging - <1> -><register>\n\n//Error registrations\nError Occurred@Acquisition - <1> >> Error Handler -><register>\nError Occurred@Logging - <1> >> Error Handler -><register>\n\n//Dynamic registrations\n// 订阅/取消订阅\n//Status@SourceModule >> API@TargetModule -><register as interrupt>\n//UrgentEvent @SourceModule >> API@TargetModule -><register as status>\n\n\n\n//Launch Acquisition Module\n"  # Data: Initialize Initialize Core Data UI: Initialize  //Permanent registrations Acquired Data@Acquisition - <1> >> Data: Update Indicators -><register> Acquired Data@Acquisition - <1> >> API: Log@Logging - <1> -><register>  //Error registrations Error Occurred@Acquisition - <1> >> Error Handler -><register> Error Occurred@Logging - <1> >> Error Handler -><register>  //Dynamic registrations // 订阅/取消订阅 //Status@SourceModule >> API@TargetModule -><register as interrupt> //UrgentEvent @SourceModule >> API@TargetModule -><register as status>    //Launch Acquisition Module
        # "#CSM \"Macro: Initialize\"\nInitialization Macro (This is called once, when the VI starts)"
        n137 = call-poly <userlib>:"Build Message with Arguments++.vi"("States With Replace Token"=w272, "<1>"=w271) -> ("States"=w270:string)  [unwired: 13 in]
        n138 = call <vilib>:"Add State(s) to Queue__JKI_lib_State_Machine.vi"("State(s) in Front (\"\")"=w270, "State(s) in (\"\")"=w275) -> ("States Out"=w274:string)  [unwired: 13 in]
      }
      frame "Macro: Start" {
        n139 = Unbundle By Name(w281) -> ("Sample Settings"=w282:T9)
        n140 = local write "温度采集开关"(TRUE ("温度采集开关")) -> ()
        n141 = call "Convert Data To API String Arguments.vim"("Data"=w282) -> ("API String"=w279:string)  [unwired: 7 in, 1 out]
        n142 = call-poly <userlib>:"Build Message with Arguments++.vi"("States With Replace Token"="API: Start >> <param> -@ Acquisition - <1>\nAPI: Start  -@ Logging - <1>" ("State"), "<param>"=w279, "<1>"=w278) -> ("States"=w276:string)  [unwired: 12 in]
        n143 = call <vilib>:"Add State(s) to Queue__JKI_lib_State_Machine.vi"("State(s) in Front (\"\")"=w276, "State(s) in (\"\")"=w284) -> ("States Out"=w283:string)  [unwired: 13 in]
      }
      frame "Macro: Stop" {
        # "#CSM \"Macro: Exit\"\nExit Macro (This is called once, when the VI exits)"
        n144 = local write "温度采集开关"(FALSE ("温度采集开关")) -> ()
        n145 = call-poly <userlib>:"Build Message with Arguments++.vi"("States With Replace Token"="//Send Message to Other CSM Modules\nAPI: Stop -@ Acquisition - <1>\nAPI: Stop -@ Logging - <1>", "<1>"=w287) -> ("States"=w285:string)  [unwired: 13 in]
        n146 = call <vilib>:"Add State(s) to Queue__JKI_lib_State_Machine.vi"("State(s) in Front (\"\")"=w285, "State(s) in (\"\")"=w291) -> ("States Out"=w290:string)  [unwired: 13 in]
      }
      frame "Macro: Exit" {
        w294 = "//Exit\nMacro: Exit-@Acquisition - <1>\nMacro: Exit-@Logging - <1>\n\n//Permanent unregistrations\nAcquired Data@Acquisition - <1> >> Data: Update Indicators -><unregister>\nAcquired Data@Acquisition - <1> >> API: Log@Logging - <1> -><unregister>\n\n//Permanent unregistrations\nError Occurred@Acquisition - <1> >> Error Handler -><unregister>\nError Occurred@Logging - <1> >> Error Handler -><unregister>\n\nData: Cleanup\nExit"  # //Exit Macro: Exit-@Acquisition - <1> Macro: Exit-@Logging - <1>  //Permanent unregistrations Acquired Data@Acquisition - <1> >> Data: Update Indicators -><unregister> Acquired Data@Acquisition - <1> >> API: Log@Logging - <1> -><unregister>  //Permanent unregistrations Error Occurred@Acquisition - <1> >> Error Handler -><unregister> Error Occurred@Logging - <1> >> Error Handler -><unregister>  Data: Cleanup Exit
        # "#CSM \"Macro: Exit\"\nExit Macro (This is called once, when the VI exits)"
        n147 = disable-structure shown="禁用" {
          frame Disabled {
            # "#NOTE\nHelper VI is equivalent to other case"
            n148 = call <userlib>:"CSM - Build Exit Messages of CSMs.vi"("State With Arguments (\"Macro: Exit“)"="Macro: Exit" ("State with Arguments(\"Macro: Exit“)"), "CSMs"=string[] ["AcquisitionTP1", "//LoggingTP1"]) -> ()  [unwired: 13 in, 1 out]
          }
          frame Enabled {
          }
        }
        n149 = call-poly <userlib>:"Build Message with Arguments++.vi"("States With Replace Token"=w294, "<1>"=w293) -> ("States"=w292:string)  [unwired: 13 in]
        n150 = call <vilib>:"Add State(s) to Queue__JKI_lib_State_Machine.vi"("State(s) in Front (\"\")"=w292, "State(s) in (\"\")"=w297) -> ("States Out"=w296:string)  [unwired: 13 in]
      }
      frame "---------- API ----------" {
        # "#CSM \"Category Seperator\"\nDo not put any code in this frame."
        n151 = call <vilib>:"Add State(s) to Queue__JKI_lib_State_Machine.vi"("State(s) in (\"\")"=w300) -> ("States Out"=w301:string)  [unwired: 14 in]
      }
      frame "API: Sample Interval" {
        # "#CSM \"Category Seperator\"\nDo not put any code in this frame."
        n152 = call "Convert API String Arguments to Data.vim"("Reference Type"=0.0, "API String"=w306) -> ("Data"=w304:dbl)  [unwired: 6 in, 1 out]
        n153 = call-poly <userlib>:"Build Message with Arguments++.vi"("States With Replace Token"="API: Sample Interval >> <param> ->| Acquisition - <1>" ("State"), "<param>"=w306, "<1>"=w309) -> ("States"=w308:string)  [unwired: 12 in]
        n154 = call <vilib>:"Add State(s) to Queue__JKI_lib_State_Machine.vi"("State(s) in Front (\"\")"=w308, "State(s) in (\"\")"=w311) -> ("States Out"=w312:string)  [unwired: 13 in]
        n155 = Bundle By Name(cluster=w307, "Sample Settings.Interval(s)"=w304) -> (w303:T11)
      }
      frame "API: Calib" {
        # "#CSM \"Category Seperator\"\nDo not put any code in this frame."
        n156 = call "Convert API String Arguments to Data.vim"("Reference Type"=dbl[] [0.0, 0.0, 0.0, 0.0, 0.0, 0.0, 0.0, 0.0] ("Calib"), "API String"=w314) -> ("Data"=w317:dbl[])  [unwired: 6 in, 1 out]
        n157 = call-poly <userlib>:"Build Message with Arguments++.vi"("States With Replace Token"="API: Sample Rate >> <param> ->| Acquisition - <1>" ("State"), "<param>"=w314, "<1>"=w319) -> ("States"=w318:string)  [unwired: 12 in]
        n158 = Bundle By Name(cluster=w316, "Sample Settings.Calib"=w317) -> (w315:T11)
        n159 = call <vilib>:"Add State(s) to Queue__JKI_lib_State_Machine.vi"("State(s) in Front (\"\")"=w318, "State(s) in (\"\")"=w321) -> ("States Out"=w322:string)  [unwired: 13 in]
      }
      frame "API: USB Port" {
        # "#CSM \"Category Seperator\"\nDo not put any code in this frame."
        n160 = call "Convert API String Arguments to Data.vim"("Reference Type"=refnum<visa-resource-name> "COM3" ("USB Port"), "API String"=w324) -> ("Data"=w327:refnum<visa-resource-name>)  [unwired: 6 in, 1 out]
        n161 = Bundle By Name(cluster=w326, "Sample Settings.USB Port"=w327) -> (w325:T11)
        n162 = call <vilib>:"Add State(s) to Queue__JKI_lib_State_Machine.vi"("State(s) in (\"\")"=w328) -> ("States Out"=w329:string)  [unwired: 14 in]
      }
    }
    n163 = Unbundle By Name(w26) -> ("子程序？"=w25:bool)
    n164 = call "State Delete.vi"("Delete?(F)"=w25, "CSM name to delete"=string[] ["Logging"], "State In"=w29) -> ("State Out"=w28:string)  [unwired: 8 in]
  }
  n165 = while {
    shift-right: [w340] -> _
    shift-left: enum16{"Idle", "Initialize", "Exit"}."Initialize" -> [w341]
    tunnel: "CSM Name" -> [w338]
    shift-right: [w336] -> _
    shift-left: w9 -> [w337]
    shift-right: [w334] -> _
    shift-left: -1 -> [w335]
    shift-right: [w333] -> _
    shift-left: _ -> [w332]
    shift-right: [w331] -> _
    shift-left: _ -> [w330]
    stop <- w339 stop-if-true
    n166 = case shown="\"Idle\", 默认" w341 {
      tunnel: [enum16{"Idle", "Initialize", "Exit"}."Idle" w359 enum16{"Idle", "Initialize", "Exit"}."Exit"] -> w340
      tunnel: [_ _ TRUE] -> w339
      tunnel: w338 -> [w345 w358 _]
      tunnel: w337 -> [w348 w356 w429]
      tunnel: [w348 w357 w429] -> w336
      tunnel: w335 -> [_ w354 _]
      tunnel: [-1 w355 _] -> w334
      tunnel: [w344 w352 _] -> w333
      tunnel: w332 -> [_ w353 w428]
      tunnel: [w342 w350 w426] -> w331
      tunnel: w330 -> [_ w351 w426]
      frame "Initialize" {
        w343 = FALSE  # your data
        n167 = call <userlib>:"CSM - Module Exit Event.vi"("Name (\"\" to Use UUID) In"=w345) -> ("CSM Exit Event"=w346:refnum<user-event>)  [unwired: 8 in, 2 out]
        n168 = register-events(w346) -> (reference out=w344:refnum<event-registration>)  [unwired: 2 in, 1 out]
        n169 = Bundle("your data"=w343) -> (w342:cluster{"your data":bool})  [unwired: 1 in]
      }
      frame "Idle", Default {
        n170 = event shown="[5] \"Chart Auto Zoom\": 值改变" {
          selector: w353 -> [_ _ _ _ _ _ _ _ _]
          dyn-events: [_ _ _ _ _ _ _ _ _] -> w352
          timeout: w354 -> [_ _ _ _ _ _ _ _ _]
          tunnel: [_ w367 enum16{"Idle", "Initialize", "Exit"}."Exit" _ _ _ _ _ _] -> w359
          tunnel: w358 -> [w361 w372 _ _ _ _ _ _ _]
          tunnel: w356 -> [w364 _ w381 w387 w396 w400 w407 w414 w423]
          tunnel: [w362 w371 w381 w388 w395 w399 w406 w413 w424] -> w357
          tunnel: [-1 _ _ _ _ _ _ _ _] -> w355
          tunnel: w351 -> [w360 w370 w379 w389 w397 w404 w411 w418 w425]
          tunnel: [w360 w370 w379 w389 w397 w404 w411 w418 w425] -> w350
          event Timeout {
            n171 = event-data() -> ()  [unwired: 1 in, 3 out]
            n172 = call-poly <userlib>:"CSM - Filter JKISM String Queue.vi"("States In"=w364) -> ("States Out"=w363:string)  [unwired: 14 in]
            n173 = call <userlib>:"CSM - Forward UI Operations to CSM.vi"("Name (\"\" to Use UUID)"=w361, "State(s) In (\"\")"=w363) -> ("States Out"=w362:string)  [unwired: 8 in, 1 out]
          }
          event Panel Close? {
            n174 = event-data() -> ()  [unwired: 1 in, 1 out]
            n175 = Two Button Dialog(message="确定关闭程序？" ("消息")) -> (T button?=w368:bool)  [unwired: 2 in]
            n176 = case shown="True" w368 {
              tunnel: w372 -> [w374 w377]
              tunnel: [w374 w376] -> w371
              tunnel: [enum16{"Idle", "Initialize", "Exit"}."Idle" enum16{"Idle", "Initialize", "Exit"}."Exit"] -> w367
              frame False {
              }
              frame True {
                n177 = call <userlib>:"CSM - Forward UI Operations to CSM.vi"("Name (\"\" to Use UUID)"=w377, "State(s) In (\"\")"="Macro: Exit" ("State")) -> ("States Out"=w376:string)  [unwired: 8 in, 1 out]
              }
            }
            n178 = event-data("Discard?"=TRUE) -> ()  [unwired: 1 in, 1 out]
          }
          event User Event {
            n179 = event-data() -> ()  [unwired: 1 in, 1 out]
          }
          event "停止": Value Change {
            n180 = event-data() -> ()  [unwired: 1 in, 1 out]
            n181 = Two Button Dialog(message="确定停止程序？" ("消息")) -> (T button?=w384:bool)  [unwired: 2 in]
            n182 = Select(t="Macro: Exit" ("State(s) in Front (\"\")"), s=w384, f="") -> (s? t:f=w382:string)
            n183 = call <vilib>:"Add State(s) to Queue__JKI_lib_State_Machine.vi"("State(s) in Front (\"\")"=w382, "State(s) in (\"\")"=w387) -> ("States Out"=w388:string)  [unwired: 13 in]
          }
          event "温度采集开关": Value Change {
            n184 = event-data() -> ()  [unwired: 1 in, 1 out]
            n185 = Select(t="Macro: Start" ("State(s) in Front (\"\")"), s="温度采集开关", f="Macro: Stop" ("State(s) in Front (\"\")")) -> (s? t:f=w390:string)
            n186 = local write "Error Occurred"(errorcluster {"status"=FALSE, "code"=0, "source"=""} ("错误常量")) -> ()
            n187 = call <vilib>:"Add State(s) to Queue__JKI_lib_State_Machine.vi"("State(s) in Front (\"\")"=w390, "State(s) in (\"\")"=w396) -> ("States Out"=w395:string)  [unwired: 13 in]
          }
          event "Chart Auto Zoom": Value Change {
            n188 = event-data() -> ()  [unwired: 1 in, 1 out]
            n189 = call "Convert Data To API String Arguments.vim"("Data"="Chart Auto Zoom") -> ("API String"=w402:string)  [unwired: 7 in, 1 out]
            n190 = call <vilib>:"Build State String with Arguments__JKI_lib_State_Machine.vi"("Arguments (\"\")"=w402, "State"="UI: Auto Zoom" ("State(s) in Front (\"\")")) -> ("State with Arguments"=w401:string)  [unwired: 4 in]
            n191 = call <vilib>:"Add State(s) to Queue__JKI_lib_State_Machine.vi"("State(s) in Front (\"\")"=w401, "State(s) in (\"\")"=w400) -> ("States Out"=w399:string)  [unwired: 13 in]
          }
          event "Interval(s)": Value Change {
            n192 = event-data() -> ()  [unwired: 1 in, 1 out]
            n193 = call "Convert Data To API String Arguments.vim"("Data"="Interval(s)") -> ("API String"=w409:string)  [unwired: 7 in, 1 out]
            n194 = call <vilib>:"Build State String with Arguments__JKI_lib_State_Machine.vi"("Arguments (\"\")"=w409, "State"="API: Sample Interval" ("State(s) in Front (\"\")")) -> ("State with Arguments"=w408:string)  [unwired: 4 in]
            n195 = call <vilib>:"Add State(s) to Queue__JKI_lib_State_Machine.vi"("State(s) in Front (\"\")"=w408, "State(s) in (\"\")"=w407) -> ("States Out"=w406:string)  [unwired: 13 in]
          }
          event "Calib": Value Change {
            n196 = event-data() -> ()  [unwired: 1 in, 1 out]
            n197 = call "Convert Data To API String Arguments.vim"("Data"="Calib") -> ("API String"=w416:string)  [unwired: 7 in, 1 out]
            n198 = call <vilib>:"Build State String with Arguments__JKI_lib_State_Machine.vi"("Arguments (\"\")"=w416, "State"="API: Calib" ("State(s) in Front (\"\")")) -> ("State with Arguments"=w415:string)  [unwired: 4 in]
            n199 = call <vilib>:"Add State(s) to Queue__JKI_lib_State_Machine.vi"("State(s) in Front (\"\")"=w415, "State(s) in (\"\")"=w414) -> ("States Out"=w413:string)  [unwired: 13 in]
          }
          event "USB Port": Value Change {
            n200 = event-data() -> ()  [unwired: 1 in, 1 out]
            n201 = call "Convert Data To API String Arguments.vim"("Data"="USB Port") -> ("API String"=w421:string)  [unwired: 7 in, 1 out]
            n202 = call <vilib>:"Build State String with Arguments__JKI_lib_State_Machine.vi"("Arguments (\"\")"=w421, "State"="API: USB Port" ("State(s) in Front (\"\")")) -> ("State with Arguments"=w419:string)  [unwired: 4 in]
            n203 = call <vilib>:"Add State(s) to Queue__jki_lib_state_machine.vi"("State(s) in Front (\"\")"=w419, "State(s) in (\"\")"=w423) -> ("States Out"=w424:string)  [unwired: 13 in]
          }
        }
      }
      frame "Exit" {
        n204 = Unregister For Events(event registration refnum=w428) -> (error out=w427:errorcluster)  [unwired: 1 in]
        n205 = call <vilib>:"Clear Errors.vi"("error in (no error)"=w427) -> ()  [unwired: 5 in, 2 out]
      }
    }
  }
  n206 = flat-sequence {
    tunnel: w5 -> [_]
    tunnel: "CSM Name" -> [w434]
    tunnel: "子程序？" -> [w432]
    frame #0 {
      n207 = Concatenate Strings("Acquisition - " ("Name(\"\" to use uuid)"), w434) -> (w436:string)
      n208 = call "Acquisition.vi"("CSM Name"=w436) -> ()  [unwired: 11 in]
      n209 = Concatenate Strings("Logging - " ("Name(\"\" to use uuid)"), w434) -> (w433:string)
      n210 = case shown="False" w432 {
        tunnel: w433 -> [w438 _]
        frame False {
          n211 = call "Logging.vi"("CSM Name"=w438) -> ()  [unwired: 11 in]
        }
        frame True {
        }
      }
    }
  }
  n212 = call <userlib>:"CSM - Sync Configuration Variables to File.vi"("All Temp Variable to Default Ini(F)"=TRUE, "error in (no error)"=w3) -> ()  [unwired: 7 in, 1 out]
